vi "WindTurbine.vi"() -> ()   [LabVIEW 2024]
panel:
  in  "Speed":u8
  out "IP":string
  out "Port":dbl
  in  "Send":bool
  # "Wind Turbine Control"
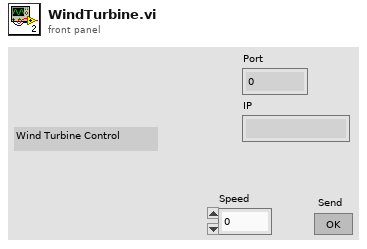
[diagram p1: front panel]
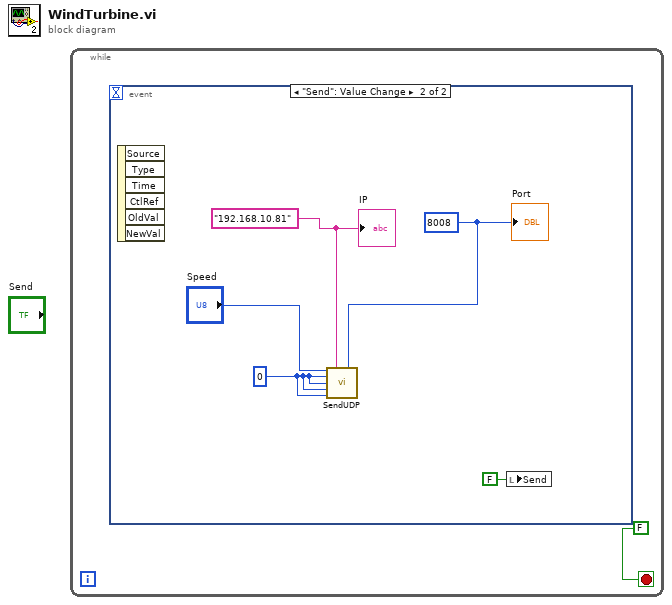
[diagram p0: block diagram]
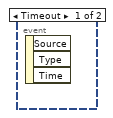
[diagram p2: hidden frame]
diagram:
  n1 = while {
    stop <- FALSE stop-if-true
    n2 = event shown="[1] \"Send\": Value Change" {
      selector: _ -> [_ _]
      dyn-events: _ -> [_ _]
      timeout: _ -> [_ _]
      event Timeout {
        n3 = event-data() -> ()  [unwired: 1 in, 3 out]
      }
      event "Send": Value Change {
        w3 = u8 0 ("Arg4")
        w5 = "192.168.10.81"
        w4 = 8008
        n4 = event-data() -> ()  [unwired: 1 in, 6 out]
        n5 = call "SendUDP.vi"("Arg3"="Speed", "IP"=w5, "Port"=w4, "Arg4"=w3, "Arg5"=w3, "Arg6"=w3, "Arg7"=w3) -> ()  [unwired: 9 in]
        n6 = local write "Send"(FALSE ("Send")) -> ()
        "Port" <- w4
        "IP" <- w5
      }
    }
  }
